vi "CE Client - Open session.vi"(5 "use TCP for local (F)":bool, 6 "error in":errorcluster, 8 "port number (3363)":u32=3363, 9 "machine name (empty - local)":string) -> (0 "error out":errorcluster, 3 "CE session out":T1={"VI refnum"=refnum, "VC Handle"=-1})   [LabVIEW 2021]
doc: "::: CalcExpress Toolkit :::\nCopyright (c) 2000-2026 Konstantin Shifershteyn. All rights reserved."
uses:
  CE Session.ctl
  vi.lib/addons/CalcExpress/cetypes.llb/VarMan Variable Context Handle.ctl
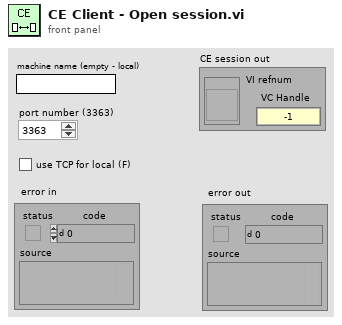
[diagram p1: front panel]
types:
  T1 = typedef "CE Session.ctl" = cluster{"VI refnum":refnum<vi>, "VC Handle":T2}
  T2 = typedef "VarMan Variable Context Handle.ctl" = i32
  T3 = enum16{"open session", "close session", "CalcExpress", "VarMan"}
  T4 = cluster{"VI refnum":refnum<vi>, "VC Handle out":i32}
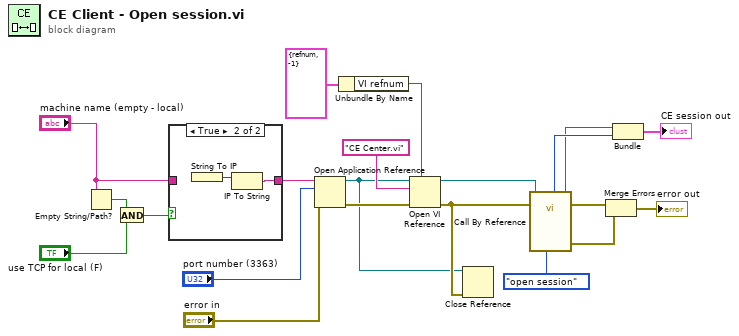
[diagram p0: block diagram]
diagram:
  n1 = Empty String/Path?(string/path="machine name (empty - local)") -> (empty?=w9:bool)
  n2 = And(x=w9, y="use TCP for local (F)") -> (x .and. y?=w7:bool)
  n3 = case shown="True" w7 {
    tunnel: [w22 w23] -> w11
    tunnel: "machine name (empty - local)" -> [w22 _]
    frame False {
    }
    frame True {
      n4 = String To IP() -> (0:w24:u32)  [unwired: 1 in]
      n5 = IP To String(2:w24) -> (0:w23:string)  [unwired: 1 in]
    }
  }
  n6 = Open Application Reference(8:"error in", 10:"port number (3363)", 11:w11) -> (0:w20:errorcluster, 3:w12:refnum<vi>)  [unwired: 1 in]
  n7 = Unbundle By Name(T1 {"VI refnum"=refnum, "VC Handle"=-1} ("CE session out")) -> ("VI refnum"=w14:refnum<vi>)
  n8 = Open VI Reference(type specifier VI Refnum (for type only)=w14, application reference (local)=w12, vi path="CE Center.vi", error in (no error)=w20) -> (vi reference=w18:refnum<vi>, error out=w17:errorcluster)  [unwired: 2 in]
  n9 = Close Reference(reference=w12, error in (no error)=w17) -> ()  [unwired: 1 out]
  n10 = call-by-ref "?"(reference=w18, error in=w17, "exec"=T3."open session") -> (reference out=w13:refnum<vi>, error out=w4:errorcluster, "error out"=w3:errorcluster, "VC Handle out"=w16:i32)  [unwired: 8 in, 1 out]
  n11 = Merge Errors(w4, w3) -> (→"error out":errorcluster)
  n12 = Bundle("VI refnum"=w13, "VC Handle out"=w16) -> (→"CE session out":T4)  [unwired: 1 in]
